vi "CIVI IDN Test.vi"() -> ()   [LabVIEW 2026]
panel:
  out "IDN Response":string
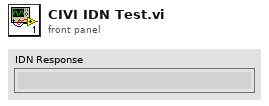
[diagram p1: front panel]
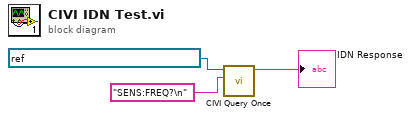
[diagram p0: block diagram]
diagram:
  n1 = call "CIVI Query Once.vi"("write buffer"="SENS:FREQ?\n", "VISA Refnum in"=refnum<visa-resource-name> "TCPIP0::127.0.0.1::5025::SOCKET" ("VISA resource name")) -> ("read buffer"=→"IDN Response":string)  [unwired: 9 in]
